vi "Close Fixture.vi"(11 "Command line args":string[](array[string])) -> (2 "Output":string, 3 "Return code":i32)   [LabVIEW 2020]
doc: "Closes the front panel of tests\\fixtures\\RemoteVI Fixture.vi (next to this VI) after aborting it if it still runs, so the fixture and the RemoteVI VIs it calls leave memory: VIPM refuses to build the package while source VIs are open, and a fixture kept in memory keeps its last values. Its connector pane is the one NI's LabVIEW CLI expects from RunVI (pattern 4815, Command line args at 11, Output at 2, Return code at 3); tools\\run-lv-integration.ps1 runs it after the suite. Return code is the error code of closing the panel."
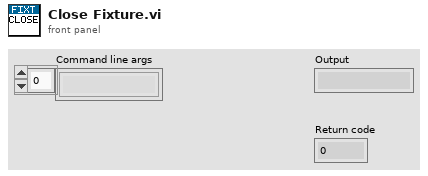
[diagram p1: front panel]
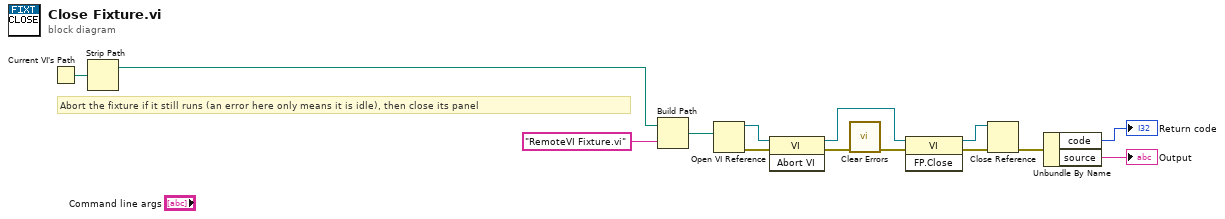
[diagram p0: block diagram]
diagram:
  # "Abort the fixture if it still runs (an error here only means it is idle), then close its panel"
  n1 = Current VI's Path() -> (path=w1:path)
  n2 = Strip Path(path=w1) -> (stripped path=w2:path)  [unwired: 1 out]
  n3 = Build Path(base path=w2, name or relative path="RemoteVI Fixture.vi") -> (appended path=w4:path)
  n4 = Open VI Reference(vi path=w4) -> (vi reference=w5:refnum<vi>, error out=w6:errorcluster)  [unwired: 5 in]
  n5 = invoke class="VI" method="Abort VI"(reference=w5, error in=w6) -> (reference out=w7:refnum<vi>, error out=w8:errorcluster)  [unwired: 1 in, 1 out]
  n6 = call <vilib>:"Clear Errors.vi"("error in (no error)"=w8) -> ("error out"=w9:errorcluster)  [unwired: 5 in, 1 out]
  n7 = invoke class="VI" method="FP.Close"(reference=w7, error in=w9) -> (reference out=w10:refnum<vi>, error out=w11:errorcluster)  [unwired: 1 in, 1 out]
  n8 = Close Reference(reference=w10, error in (no error)=w11) -> (error out=w12:errorcluster)
  n9 = Unbundle By Name(w12) -> ("code"=→"Return code":i32, "source"=→"Output":string)
